vi "set Start and Stop Frequency.vi"(8 "error in (no error)":errorcluster, 10 "Start/Stop Frequency(Hz)":T1 {"Stop" format="%#_6p"; "Start" format="%#_6p"}, 11 "Keysight 9020A in":refnum<class "Keysight 9020A.lvclass">) -> (0 "error out":errorcluster, 3 "Keysight 9020A out":refnum<class "Keysight 9020A.lvclass">)   [LabVIEW 2023, in "Spectrum Analyzer.lvlib" / "Keysight 9020A.lvclass"]
uses:
  Keysight 9020A.lvclass
  TYPE DEFINITION/TYPE Start and Stop Frequency.ctl
  Keysight 9020A.lvclass/Keysight 9020A.ctl
  Spectrum Analyzer.lvlib
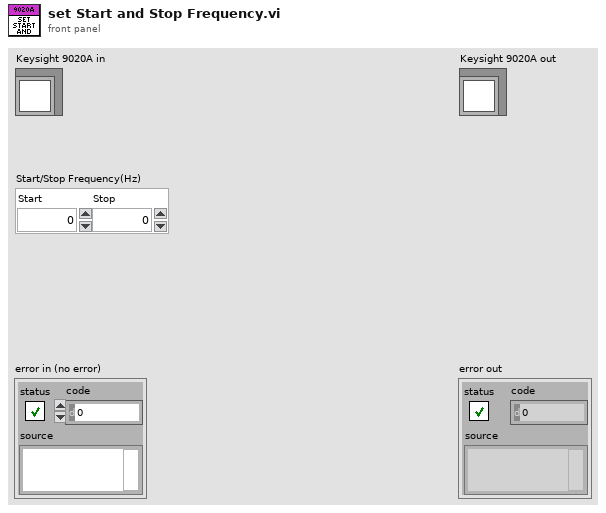
[diagram p1: front panel]
types:
  T1 = typedef "Spectrum Analyzer.lvlib/TYPE Start and Stop Frequency.ctl" = cluster{"Start":dbl, "Stop":dbl}
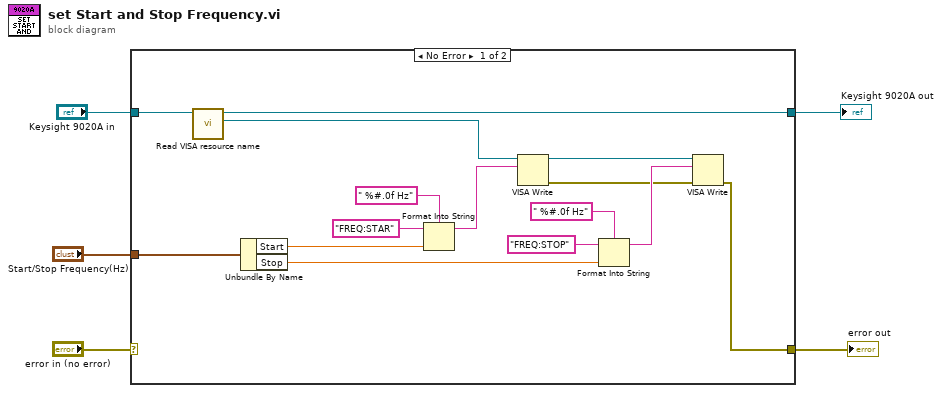
[diagram p0: block diagram]
diagram:
  n1 = case shown="No Error" "error in (no error)" {
    selector: "error in (no error)" -> [_ w21]
    tunnel: "Keysight 9020A in" -> [w20 w22]
    tunnel: [w19 w22] -> w4
    tunnel: [w6 w21] -> w2
    tunnel: "Start/Stop Frequency(Hz)" -> [w15 _]
    frame No Error {
      n2 = call "Read VISA resource name.vi"("Keysight 9020A in"=w20) -> ("VISA resource name"=w17:refnum<visa-resource-name>, "Keysight 9020A out"=w19:refnum<class "Keysight 9020A.lvclass">)  [unwired: 8 in, 1 out]
      n3 = Unbundle By Name(w15) -> ("Start"=w13:dbl, "Stop"=w8:dbl)
      n4 = Format Into String(format string=" %#.0f Hz", initial string="FREQ:STAR", w13) -> (resulting string=w16:string)  [unwired: 1 in, 1 out]
      n5 = VISA Write(VISA resource name=w17, write buffer=w16) -> (VISA resource name out=w9:refnum<visa-resource-name>, error out=w7:errorcluster)  [unwired: 1 in, 1 out]
      n6 = Format Into String(format string=" %#.0f Hz", initial string="FREQ:STOP", w8) -> (resulting string=w11:string)  [unwired: 1 in, 1 out]
      n7 = VISA Write(VISA resource name=w9, write buffer=w11, error in (no error)=w7) -> (error out=w6:errorcluster)  [unwired: 2 out]
    }
    frame Error {
    }
  }
  "error out" <- w2
  "Keysight 9020A out" <- w4
